vi "RemoteVI Show Status.vi"(11 "error in":errorcluster) -> (15 "error out":errorcluster)   [LabVIEW 2020, in "RemoteVI.lvlib"]
doc: "Opens the RemoteVI Status window (RemoteVI Status Panel.vi, found next to this VI) and returns at once: if it is already open it is brought to the front, else it is opened and run. Put it behind a button or a menu item of your application to see what RemoteVI shares, who is connected and how fast frames go out. Closing that window stops no share."
uses:
  RemoteVI.lvlib
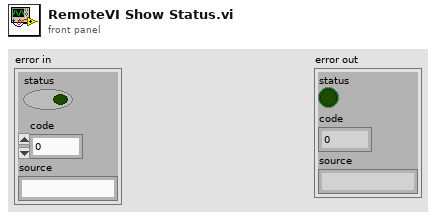
[diagram p1: front panel]
types:
  T1 = enum32{"Bad", "Idle", "Run top level", "Running"}
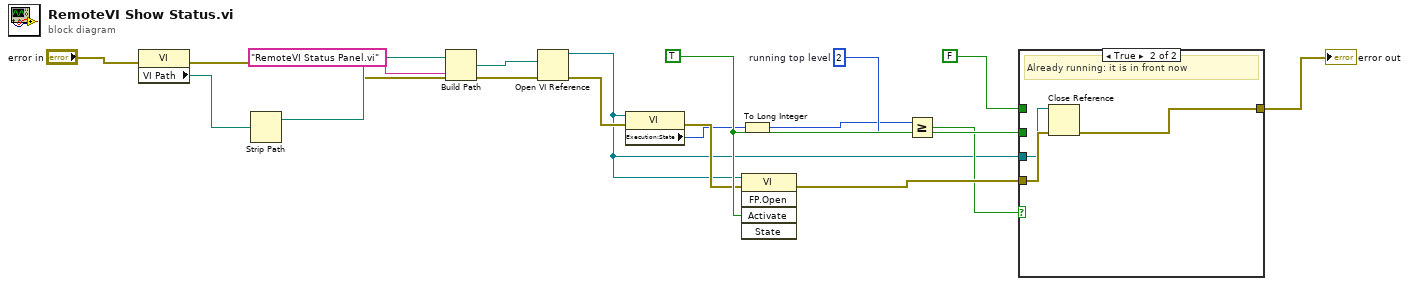
[diagram p0: block diagram]
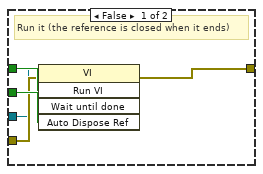
[diagram p2: hidden frame]
diagram:
  w14 = TRUE
  w12 = 2  # running top level
  n1 = property class="VI"(error in="error in") -> (error out=w2:errorcluster, "VI Path"=w3:path)  [unwired: 1 in, 1 out]
  n2 = Strip Path(path=w3) -> (stripped path=w4:path)  [unwired: 1 out]
  n3 = Build Path(base path=w4, name or relative path="RemoteVI Status Panel.vi") -> (appended path=w6:path)
  n4 = Open VI Reference(vi path=w6, error in (no error)=w2) -> (vi reference=w7:refnum<vi>, error out=w8:errorcluster)  [unwired: 4 in]
  n5 = property class="VI"(reference=w7, error in=w8) -> (error out=w10:errorcluster, "Execution:State"=w9:T1)  [unwired: 1 out]
  n6 = To Long Integer(number=w9) -> (32bit integer=w11:i32)
  n7 = invoke class="VI" method="FP.Open"(reference=w7, error in=w10, "Activate"=w14) -> (error out=w16:errorcluster)  [unwired: 2 in, 4 out]
  n8 = Greater Or Equal?(x=w11, y=w12) -> (x >= y?=w13:bool)
  n9 = case shown="True" w13 {
    tunnel: FALSE -> [w20 _]
    tunnel: w14 -> [w21 _]
    tunnel: w7 -> [w18 w23]
    tunnel: w16 -> [w19 w24]
    tunnel: [w22 w25] -> w17
    frame False {
      # "Run it (the reference is closed when it ends)"
      n10 = invoke class="VI" method="Run VI"(reference=w18, error in=w19, "Wait until done"=w20, "Auto Dispose Ref"=w21) -> (error out=w22:errorcluster)  [unwired: 1 in, 4 out]
    }
    frame True {
      # "Already running: it is in front now"
      n11 = Close Reference(reference=w23, error in (no error)=w24) -> (error out=w25:errorcluster)
    }
  }
  "error out" <- w17
